vi "Test List Folder.vi"(8 "error in (no error)":errorcluster) -> (0 "error out":errorcluster, 3 "Pass?":bool)   [LabVIEW 2020]
uses:
  G-Unicode/Types/UTF-8 String/UTF-8 String.lvclass
  G-Unicode/Unicode/Controls/String Encoding.ctl
  G-Unicode/Types/UTF-8 String/UTF-8 String.lvclass/UTF-8 String.ctl
  G-Unicode/Types/UTF-8 Path/UTF-8 Path.lvclass/UTF-8 Path.ctl
  a54f53b9-e182-45f2-9df3-3ad09404b159.vi
  723a0a90-94e1-4b00-9b8e-63d3f230976f.vi
  2400d2f7-f357-4396-a7fa-e5c669c64687.vi
  2b28c85d-6eb6-42f1-9791-7ceb4d579ff7.vi
  8ef4e441-2967-427c-b2f5-611982e59b74.vi
  d10c2814-85e2-4189-8dec-6298f27de2e3.vi
  570365af-4a81-404b-8e59-15630106fe67.vi
  ef45a9f8-57a2-414a-8a1b-10db4b84396b.vi
  eeafece5-71ef-472f-ba41-926d6844275a.vi
  410ed48b-bd58-4d2b-973d-16e07af476d5.vi
  G-Unicode/Private/Conversion/Text as Encoded Path.vi
  G-Unicode/Private/Conversion/Polymorphic VIs/Text as Encoded Path (LabVIEW Path).vi
  G-Unicode/Types/UTF-8 Path/Write Encoded UTF-8 Path.vi
  G-Unicode/Private/Conversion/Path as Encoded Path.vi
  G-Unicode/Private/Conversion/Polymorphic VIs/Path as Encoded Path (LabVIEW Path).vi
  G-Unicode/Unicode/Encode String.vi
  723a0a90-94e1-4b00-9b8e-63d3f230976f.vi/46bf550a-28c6-4dfd-813a-9b0ad34779ef.vi
  G-Unicode/Private/Conversion/String as Encoded String.vi
  G-Unicode/Private/Conversion/Polymorphic VIs/String as Encoded String (UTF-8 String).vi
  G-Unicode/Types/UTF-8 String/Write Encoded UTF-8 String.vi
  G-Unicode/Private/Conversion/Path as UTF-8 Path.vi
  G-Unicode/Private/Conversion/Polymorphic VIs/Path as UTF-8 Path (UTF-8 Path).vi
  2400d2f7-f357-4396-a7fa-e5c669c64687.vi/5269e09c-4216-478e-8686-9fb7d38e224a.vi
  2400d2f7-f357-4396-a7fa-e5c669c64687.vi/d1f4a45d-6f02-44dd-a40b-2b28d80e6519.vi
  G-Unicode/Private/Library/gu_list_folder.vi
  2400d2f7-f357-4396-a7fa-e5c669c64687.vi/8eb4f0ed-0012-4550-978e-be3f7301df70.vi
  2400d2f7-f357-4396-a7fa-e5c669c64687.vi/f7e6584c-01ed-423f-9bcd-660954191d0d.vi
  G-Unicode/Private/Conversion/Polymorphic VIs/Text as Encoded Path (UTF-8 String).vi
  G-Unicode/Private/Conversion/Polymorphic VIs/Path as Encoded Path (UTF-8 Path).vi
  8ef4e441-2967-427c-b2f5-611982e59b74.vi/5269e09c-4216-478e-8686-9fb7d38e224a.vi
  8ef4e441-2967-427c-b2f5-611982e59b74.vi/d1f4a45d-6f02-44dd-a40b-2b28d80e6519.vi
  8ef4e441-2967-427c-b2f5-611982e59b74.vi/8eb4f0ed-0012-4550-978e-be3f7301df70.vi
  8ef4e441-2967-427c-b2f5-611982e59b74.vi/f7e6584c-01ed-423f-9bcd-660954191d0d.vi
  570365af-4a81-404b-8e59-15630106fe67.vi/c24c063b-f849-48a1-b323-238a063d7118.vi
  570365af-4a81-404b-8e59-15630106fe67.vi/a2fd6c11-d594-45c9-8624-1f0a1df69df3.vi
  570365af-4a81-404b-8e59-15630106fe67.vi/1fd3173e-d32e-42cb-8f0d-819132eb8e27.vi
  570365af-4a81-404b-8e59-15630106fe67.vi/bb7c39fc-ad8e-447d-bc50-468674bfb562.vi
  ef45a9f8-57a2-414a-8a1b-10db4b84396b.vi/3a31b270-3bb6-4c58-a256-c5fcc2c98f09.vi
  ef45a9f8-57a2-414a-8a1b-10db4b84396b.vi/0ec5df2d-ef9b-4f84-a6a8-ffcedd45c4dc.vi
  G-Unicode/Private/Conversion/Polymorphic VIs/Path as UTF-8 Path (LabVIEW Path).vi
  eeafece5-71ef-472f-ba41-926d6844275a.vi/5269e09c-4216-478e-8686-9fb7d38e224a.vi
  eeafece5-71ef-472f-ba41-926d6844275a.vi/d1f4a45d-6f02-44dd-a40b-2b28d80e6519.vi
  eeafece5-71ef-472f-ba41-926d6844275a.vi/8eb4f0ed-0012-4550-978e-be3f7301df70.vi
  eeafece5-71ef-472f-ba41-926d6844275a.vi/f7e6584c-01ed-423f-9bcd-660954191d0d.vi
  G-Unicode/Private/Conversion/Polymorphic VIs/String as Encoded String (LabVIEW String).vi
  410ed48b-bd58-4d2b-973d-16e07af476d5.vi/5269e09c-4216-478e-8686-9fb7d38e224a.vi
  410ed48b-bd58-4d2b-973d-16e07af476d5.vi/d1f4a45d-6f02-44dd-a40b-2b28d80e6519.vi
  410ed48b-bd58-4d2b-973d-16e07af476d5.vi/8eb4f0ed-0012-4550-978e-be3f7301df70.vi
  410ed48b-bd58-4d2b-973d-16e07af476d5.vi/f7e6584c-01ed-423f-9bcd-660954191d0d.vi
  G-Unicode/Private/Conversion/Text to UTF-8.vi
  G-Unicode/Private/Conversion/Polymorphic VIs/Text to UTF-8 (LabVIEW Path).vi
  G-Unicode/Unicode/Detect String Encoding.vi
  G-Unicode/Private/Conversion/Polymorphic VIs/Text to UTF-8 (LabVIEW String).vi
  G-Unicode/Private/Conversion/Encoded UTF-8 String to Encoded UTF-16LE String.vi
  G-Unicode/Unicode/SubVIs/UTF-16 Byte Swap.vi
  G-Unicode/Private/Conversion/UTF-8 to Text.vi
  G-Unicode/Private/Conversion/Polymorphic VIs/UTF-8 to Text (LabVIEW String).vi
  G-Unicode/Private/Conversion/Encoded UTF-16LE String to Encoded UTF-8 String.vi
  G-Unicode/Unicode/Prepend BOM.vi
  2400d2f7-f357-4396-a7fa-e5c669c64687.vi/5269e09c-4216-478e-8686-9fb7d38e224a.vi/c24c063b-f849-48a1-b323-238a063d7118.vi
  2400d2f7-f357-4396-a7fa-e5c669c64687.vi/5269e09c-4216-478e-8686-9fb7d38e224a.vi/a2fd6c11-d594-45c9-8624-1f0a1df69df3.vi
  2400d2f7-f357-4396-a7fa-e5c669c64687.vi/5269e09c-4216-478e-8686-9fb7d38e224a.vi/1fd3173e-d32e-42cb-8f0d-819132eb8e27.vi
  2400d2f7-f357-4396-a7fa-e5c669c64687.vi/5269e09c-4216-478e-8686-9fb7d38e224a.vi/bb7c39fc-ad8e-447d-bc50-468674bfb562.vi
  G-Unicode/Private/Conversion/Text as Encoded String.vi
  G-Unicode/Private/Conversion/Polymorphic VIs/Text as Encoded String (UTF-8 Path).vi
  G-Unicode/Private/Library/Result To Error.vi
  2400d2f7-f357-4396-a7fa-e5c669c64687.vi/8eb4f0ed-0012-4550-978e-be3f7301df70.vi/3a31b270-3bb6-4c58-a256-c5fcc2c98f09.vi
  2400d2f7-f357-4396-a7fa-e5c669c64687.vi/8eb4f0ed-0012-4550-978e-be3f7301df70.vi/0ec5df2d-ef9b-4f84-a6a8-ffcedd45c4dc.vi
  G-Unicode/Private/Conversion/Text as String.vi
  G-Unicode/Private/Conversion/Polymorphic VIs/Text as String (UTF-8 Path).vi
  G-Unicode/Types/UTF-8 Path/Read Encoded UTF-8 Path.vi
  8ef4e441-2967-427c-b2f5-611982e59b74.vi/5269e09c-4216-478e-8686-9fb7d38e224a.vi/c24c063b-f849-48a1-b323-238a063d7118.vi
  8ef4e441-2967-427c-b2f5-611982e59b74.vi/5269e09c-4216-478e-8686-9fb7d38e224a.vi/a2fd6c11-d594-45c9-8624-1f0a1df69df3.vi
  8ef4e441-2967-427c-b2f5-611982e59b74.vi/5269e09c-4216-478e-8686-9fb7d38e224a.vi/1fd3173e-d32e-42cb-8f0d-819132eb8e27.vi
  8ef4e441-2967-427c-b2f5-611982e59b74.vi/5269e09c-4216-478e-8686-9fb7d38e224a.vi/bb7c39fc-ad8e-447d-bc50-468674bfb562.vi
  8ef4e441-2967-427c-b2f5-611982e59b74.vi/8eb4f0ed-0012-4550-978e-be3f7301df70.vi/3a31b270-3bb6-4c58-a256-c5fcc2c98f09.vi
  8ef4e441-2967-427c-b2f5-611982e59b74.vi/8eb4f0ed-0012-4550-978e-be3f7301df70.vi/0ec5df2d-ef9b-4f84-a6a8-ffcedd45c4dc.vi
  G-Unicode/Private/Library/gu_string_subset.vi
  G-Unicode/Private/Library/gu_to_lower_case.vi
  G-Unicode/Private/Library/gu_search_split_string.vi
  G-Unicode/Private/Conversion/Polymorphic VIs/Text as Encoded String (UTF-8 String).vi
  G-Unicode/Types/UTF-8 Path/New UTF-8 Path.vi
  eeafece5-71ef-472f-ba41-926d6844275a.vi/5269e09c-4216-478e-8686-9fb7d38e224a.vi/c24c063b-f849-48a1-b323-238a063d7118.vi
  eeafece5-71ef-472f-ba41-926d6844275a.vi/5269e09c-4216-478e-8686-9fb7d38e224a.vi/a2fd6c11-d594-45c9-8624-1f0a1df69df3.vi
  eeafece5-71ef-472f-ba41-926d6844275a.vi/5269e09c-4216-478e-8686-9fb7d38e224a.vi/1fd3173e-d32e-42cb-8f0d-819132eb8e27.vi
  eeafece5-71ef-472f-ba41-926d6844275a.vi/5269e09c-4216-478e-8686-9fb7d38e224a.vi/bb7c39fc-ad8e-447d-bc50-468674bfb562.vi
  eeafece5-71ef-472f-ba41-926d6844275a.vi/8eb4f0ed-0012-4550-978e-be3f7301df70.vi/3a31b270-3bb6-4c58-a256-c5fcc2c98f09.vi
  eeafece5-71ef-472f-ba41-926d6844275a.vi/8eb4f0ed-0012-4550-978e-be3f7301df70.vi/0ec5df2d-ef9b-4f84-a6a8-ffcedd45c4dc.vi
  410ed48b-bd58-4d2b-973d-16e07af476d5.vi/5269e09c-4216-478e-8686-9fb7d38e224a.vi/c24c063b-f849-48a1-b323-238a063d7118.vi
  410ed48b-bd58-4d2b-973d-16e07af476d5.vi/5269e09c-4216-478e-8686-9fb7d38e224a.vi/a2fd6c11-d594-45c9-8624-1f0a1df69df3.vi
  410ed48b-bd58-4d2b-973d-16e07af476d5.vi/5269e09c-4216-478e-8686-9fb7d38e224a.vi/1fd3173e-d32e-42cb-8f0d-819132eb8e27.vi
  410ed48b-bd58-4d2b-973d-16e07af476d5.vi/5269e09c-4216-478e-8686-9fb7d38e224a.vi/bb7c39fc-ad8e-447d-bc50-468674bfb562.vi
  410ed48b-bd58-4d2b-973d-16e07af476d5.vi/8eb4f0ed-0012-4550-978e-be3f7301df70.vi/3a31b270-3bb6-4c58-a256-c5fcc2c98f09.vi
  410ed48b-bd58-4d2b-973d-16e07af476d5.vi/8eb4f0ed-0012-4550-978e-be3f7301df70.vi/0ec5df2d-ef9b-4f84-a6a8-ffcedd45c4dc.vi
  G-Unicode/Unicode/Strip BOM.vi
  G-Unicode/Unicode/Detect String Encoding.vi/f4e2713d-ca87-487a-b901-d606fc3002c3.vi
  G-Unicode/Unicode/SubVIs/Byte Order Marks.vi
  G-Unicode/Unicode/Detect BOM.vi
  G-Unicode/Private/Conversion/Polymorphic VIs/Text as Encoded String (LabVIEW String).vi
  G-Unicode/Private/Memory/Copy String.vi
  G-Unicode/Private/Memory/Copy String.vi/4d47babd-4a2d-4eb7-b91b-7e707d692665.vi
  G-Unicode/Private/Library/gu_free.vi
  G-Unicode/Private/Library/gu_is_text_utf16.vi
  G-Unicode/Private/Library/gu_is_text_utf8.vi
  <vilib>/Utility/error.llb/Error Cluster From Error Code.vi
  G-Unicode/Private/Memory/Copy String Array.vi
  G-Unicode/File IO/Path to Short Name (Unicode).vi
  G-Unicode/Types/UTF-8 Path/UTF-8 Path.lvclass
  G-Unicode/G-Unicode.lvlib
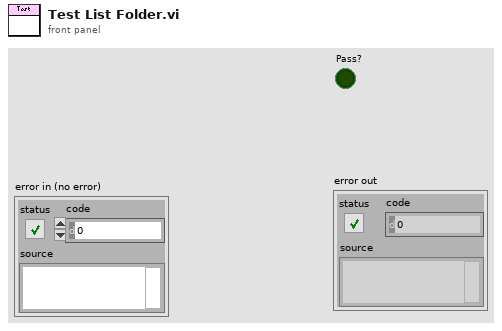
[diagram p1: front panel]
types:
  T1 = typedef "G-Unicode.lvlib/String Encoding.ctl" = enum16{"ANSI", "UTF-8", "UTF-16LE", "UTF-16BE", "Unknown"}
  T2 = typedef "G-Unicode.lvlib/Encoded UTF-8 String.ctl" = string
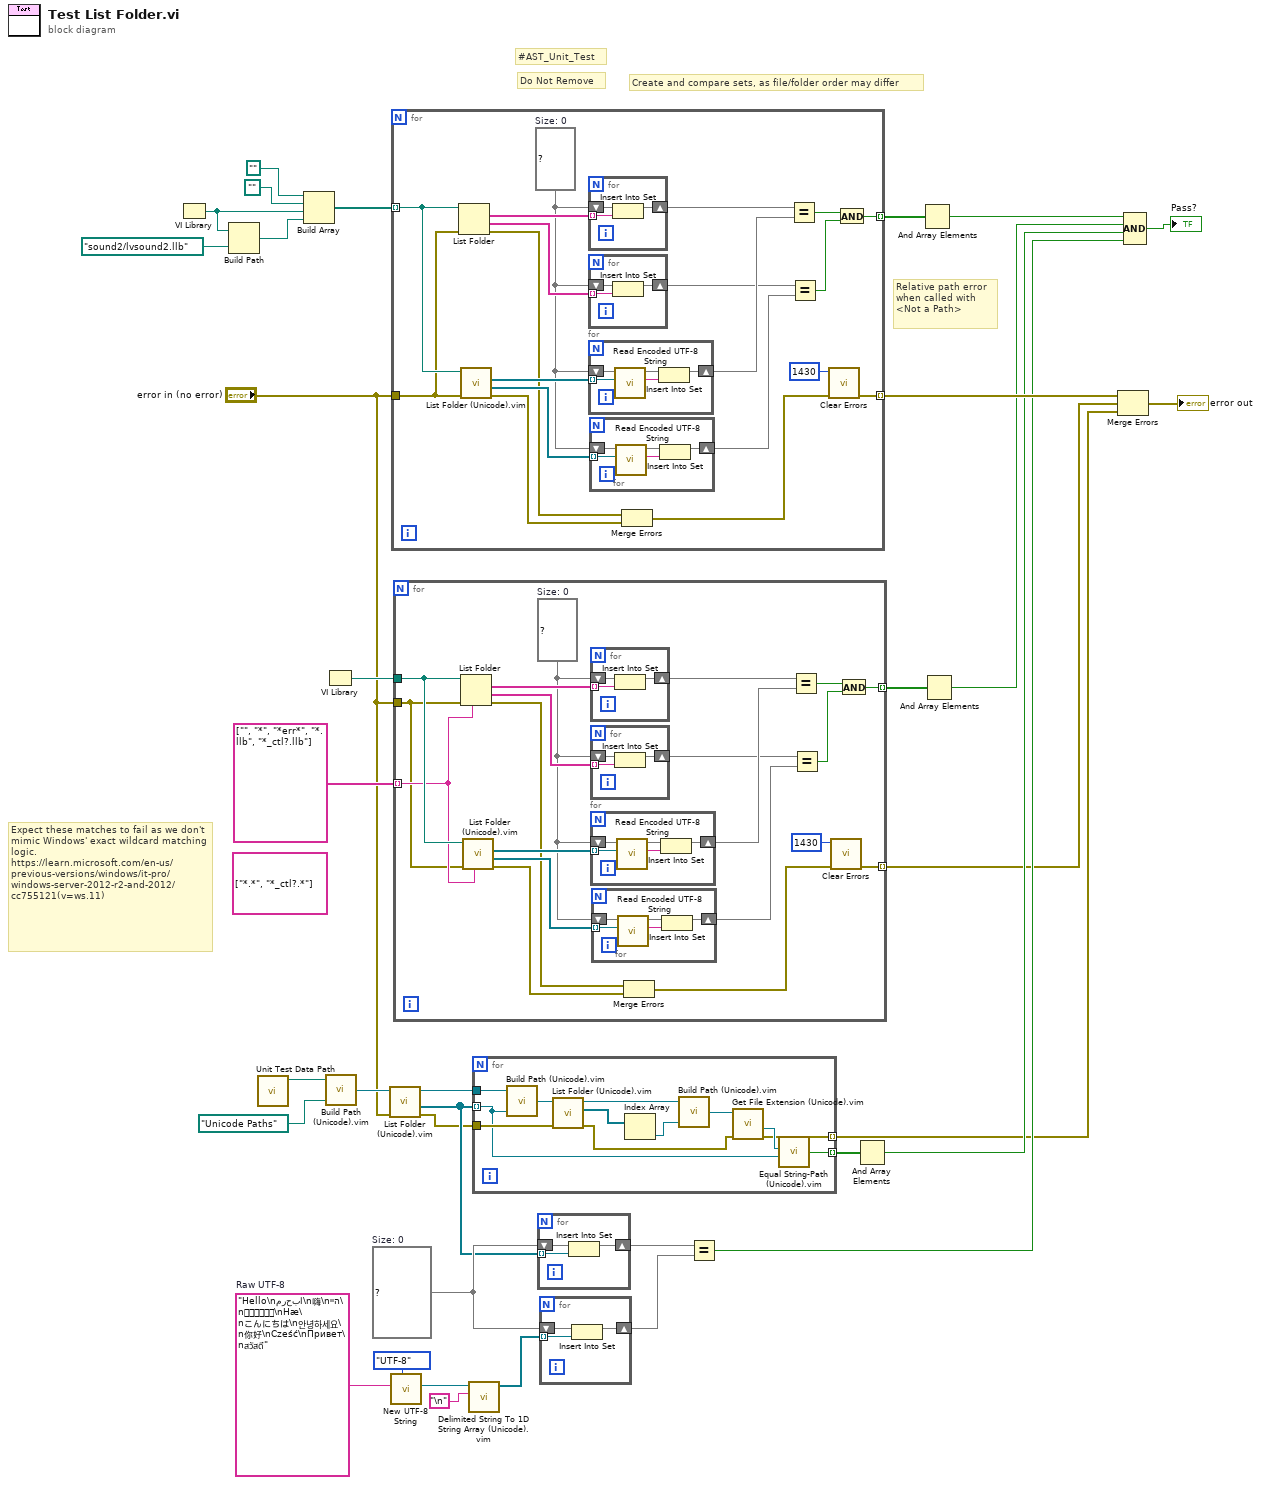
[diagram p0: block diagram]
diagram:
  (unwired) string[] ["*.*", "*_ctl?.*"]
  w28 = set{refnum<class "UTF-8 String.lvclass">} {}  # Size: 0
  w2 = "Hello\nمرحبا\n嗨\nהיי\nनमस्ते\nHæ\nこんにちは\n안녕하세요\n你好\nCześć\nПривет\nสวัสดี"  # Raw UTF-8
  # "Expect these matches to fail as we don't mimic Windows' exact wildcard matching logic.\nhttps://learn.microsoft.com/en-us/previous-versions/windows/it-pro/windows-server-2012-r2-and-2012/cc755121(v=ws.11)"
  # "Create and compare sets, as file/folder order may differ"
  # "Relative path error when called with <Not a Path>"
  # "Do Not Remove"
  # "#AST_Unit_Test"
  n1 = VI Library() -> (path=w14:path)
  n2 = Build Path(base path=w14, name or relative path=path "sound2/lvsound2.llb") -> (appended path=w15:path)
  n3 = call "Unit Test Data Path.vi"() -> ("Test Data Path"=w23:path)  [unwired: 11 in]
  n4 = Build Array(path "", path "", w14, w15) -> (w33:path[])
  n5 = VI Library() -> (path=w12:path)
  n6 = call "Build Path (Unicode).vim"("Base Path"=w23, "Name or Relative Path"=path "Unicode Paths") -> ("Appended Path"=w22:refnum<class "UTF-8 Path.lvclass">)  [unwired: 6 in, 1 out]
  n7 = call "List Folder (Unicode).vim"("error in"="error in (no error)", "Path"=w22) -> ("error out"=w7:errorcluster, "Folder Names"=w20:refnum<class "UTF-8 String.lvclass">[], "Path Out"=w19:refnum<class "UTF-8 Path.lvclass">)  [unwired: 6 in, 1 out]
  n8 = call "New UTF-8 String.vi"("Input Encoding (ANSI)"=String_Encoding."UTF-8", "String"=w2) -> ("UTF-8 String"=w4:refnum<class "UTF-8 String.lvclass">)  [unwired: 8 in, 1 out]
  n9 = for {
    tunnel: w33 -> [w54] mode=indexing
    tunnel: [w41] -> w35 mode=indexing
    tunnel: "error in (no error)" -> [w51]
    tunnel: [w37] -> w34 mode=indexing
    w48 = set{string} {}  # Size: 0
    n10 = List Folder(path=w54, error in=w51) -> (filenames=w53:string[], folder names=w52:string[], error out=w40:errorcluster)  [unwired: 2 in, 1 out]
    n11 = call "List Folder (Unicode).vim"("error in"=w51, "Path"=w54) -> ("error out"=w39:errorcluster, "Folder Names"=w49:refnum<class "UTF-8 String.lvclass">[], "Filenames"=w50:refnum<class "UTF-8 String.lvclass">[])  [unwired: 6 in, 1 out]
    n12 = for {
      tunnel: w53 -> [w68] mode=indexing
      shift-right: [w66] -> w47
      shift-left: w48 -> [w67]
      n13 = Insert Into Set(10:w68, 11:w67) -> (3:w66:set{string})  [unwired: 1 out]
    }
    n14 = for {
      tunnel: w52 -> [w65] mode=indexing
      shift-right: [w63] -> w45
      shift-left: w48 -> [w64]
      n15 = Insert Into Set(10:w65, 11:w64) -> (3:w63:set{string})  [unwired: 1 out]
    }
    n16 = for {
      tunnel: w50 -> [w60] mode=indexing
      shift-right: [w61] -> w46
      shift-left: w48 -> [w62]
      n17 = call "Read Encoded UTF-8 String.vi"("UTF-8 String"=w60) -> ("Encoded UTF-8 String"=w59:T2)  [unwired: 10 in]
      n18 = Insert Into Set(10:w59, 11:w62) -> (3:w61:set{string})  [unwired: 1 out]
    }
    n19 = for {
      tunnel: w49 -> [w56] mode=indexing
      shift-right: [w57] -> w44
      shift-left: w48 -> [w58]
      n20 = call "Read Encoded UTF-8 String.vi"("UTF-8 String"=w56) -> ("Encoded UTF-8 String"=w55:T2)  [unwired: 10 in]
      n21 = Insert Into Set(10:w55, 11:w58) -> (3:w57:set{string})  [unwired: 1 out]
    }
    n22 = Merge Errors(w40, w39) -> (w38:errorcluster)
    n23 = Equal?(x=w47, y=w46) -> (x = y?=w43:bool)
    n24 = Equal?(x=w45, y=w44) -> (x = y?=w42:bool)
    n25 = call <vilib>:"Clear Errors.vi"("error in (no error)"=w38, "specific error code to clear (0: all)"=1430) -> ("error out"=w37:errorcluster)  [unwired: 4 in, 1 out]
    n26 = And(x=w43, y=w42) -> (x .and. y?=w41:bool)
  }
  n27 = for {
    tunnel: w12 -> [w88]
    tunnel: [w76] -> w13 mode=indexing
    tunnel: [w72] -> w9 mode=indexing
    tunnel: string[] ["", "*", "*err*", "*.llb", "*_ctl?.llb"] -> [w70] mode=indexing
    tunnel: "error in (no error)" -> [w69]
    w83 = set{string} {}  # Size: 0
    n28 = List Folder(path=w88, pattern=w70, error in=w69) -> (filenames=w87:string[], folder names=w86:string[], error out=w75:errorcluster)  [unwired: 1 in, 1 out]
    n29 = call "List Folder (Unicode).vim"("Pattern"=w70, "error in"=w69, "Path"=w88) -> ("error out"=w74:errorcluster, "Folder Names"=w84:refnum<class "UTF-8 String.lvclass">[], "Filenames"=w85:refnum<class "UTF-8 String.lvclass">[])  [unwired: 5 in, 1 out]
    n30 = for {
      tunnel: w87 -> [w102] mode=indexing
      shift-right: [w100] -> w82
      shift-left: w83 -> [w101]
      n31 = Insert Into Set(10:w102, 11:w101) -> (3:w100:set{string})  [unwired: 1 out]
    }
    n32 = for {
      tunnel: w86 -> [w99] mode=indexing
      shift-right: [w97] -> w80
      shift-left: w83 -> [w98]
      n33 = Insert Into Set(10:w99, 11:w98) -> (3:w97:set{string})  [unwired: 1 out]
    }
    n34 = for {
      tunnel: w85 -> [w94] mode=indexing
      shift-right: [w95] -> w81
      shift-left: w83 -> [w96]
      n35 = call "Read Encoded UTF-8 String.vi"("UTF-8 String"=w94) -> ("Encoded UTF-8 String"=w93:T2)  [unwired: 10 in]
      n36 = Insert Into Set(10:w93, 11:w96) -> (3:w95:set{string})  [unwired: 1 out]
    }
    n37 = for {
      tunnel: w84 -> [w90] mode=indexing
      shift-right: [w91] -> w79
      shift-left: w83 -> [w92]
      n38 = call "Read Encoded UTF-8 String.vi"("UTF-8 String"=w90) -> ("Encoded UTF-8 String"=w89:T2)  [unwired: 10 in]
      n39 = Insert Into Set(10:w89, 11:w92) -> (3:w91:set{string})  [unwired: 1 out]
    }
    n40 = Merge Errors(w75, w74) -> (w73:errorcluster)
    n41 = Equal?(x=w82, y=w81) -> (x = y?=w78:bool)
    n42 = Equal?(x=w80, y=w79) -> (x = y?=w77:bool)
    n43 = call <vilib>:"Clear Errors.vi"("error in (no error)"=w73, "specific error code to clear (0: all)"=1430) -> ("error out"=w72:errorcluster)  [unwired: 4 in, 1 out]
    n44 = And(x=w78, y=w77) -> (x .and. y?=w76:bool)
  }
  n45 = call "Delimited String To 1D String Array (Unicode).vim"("Delimiter (tab)"="\n", "Delimited String"=w4) -> ("String Array"=w1:refnum<class "UTF-8 String.lvclass">[])  [unwired: 8 in, 1 out]
  n46 = for {
    tunnel: w20 -> [w103] mode=indexing
    tunnel: w19 -> [w114]
    tunnel: [w107] -> w18 mode=indexing
    tunnel: w7 -> [w106]
    tunnel: [w104] -> w8 mode=indexing
    n47 = call "Build Path (Unicode).vim"("Base Path"=w114, "Name or Relative Path"=w103) -> ("Appended Path"=w113:refnum<class "UTF-8 Path.lvclass">)  [unwired: 6 in, 1 out]
    n48 = call "List Folder (Unicode).vim"("error in"=w106, "Path"=w113) -> ("error out"=w105:errorcluster, "Filenames"=w112:refnum<class "UTF-8 String.lvclass">[], "Path Out"=w111:refnum<class "UTF-8 Path.lvclass">)  [unwired: 6 in, 1 out]
    n49 = Index Array(array=w112) -> (element=w110:refnum<class "UTF-8 String.lvclass">)  [unwired: 1 in]
    n50 = call "Build Path (Unicode).vim"("Base Path"=w111, "Name or Relative Path"=w110) -> ("Appended Path"=w109:refnum<class "UTF-8 Path.lvclass">)  [unwired: 6 in, 1 out]
    n51 = call "Get File Extension (Unicode).vim"("error in (no error)"=w105, "file"=w109) -> ("error out"=w104:errorcluster, "filename without extension"=w108:refnum<class "UTF-8 String.lvclass">)  [unwired: 5 in, 3 out]
    n52 = call "Equal String-Path (Unicode).vim"("y"=w103, "x"=w108) -> ("Equal?"=w107:bool)  [unwired: 7 in, 1 out]
  }
  n53 = for {
    tunnel: w20 -> [w115] mode=indexing
    shift-right: [w116] -> w27
    shift-left: w28 -> [w117]
    n54 = Insert Into Set(10:w115, 11:w117) -> (3:w116:set{refnum<class "UTF-8 String.lvclass">})  [unwired: 1 out]
  }
  n55 = for {
    shift-right: [w119] -> w26
    shift-left: w28 -> [w120]
    tunnel: w1 -> [w118] mode=indexing
    n56 = Insert Into Set(10:w118, 11:w120) -> (3:w119:set{refnum<class "UTF-8 String.lvclass">})  [unwired: 1 out]
  }
  n57 = Equal?(x=w27, y=w26) -> (x = y?=w17:bool)
  n58 = And Array Elements(Boolean array=w18) -> (logical AND=w16:bool)
  n59 = And Array Elements(Boolean array=w35) -> (logical AND=w25:bool)
  n60 = And Array Elements(Boolean array=w13) -> (logical AND=w10:bool)
  n61 = Merge Errors(w34, w9, w8) -> (→"error out":errorcluster)
  n62 = Compound Arithmetic op=AND(w25, w10, w16, w17) -> (→"Pass?":bool)
